vi "Check DAQmx Installed.vi"() -> (3 "DAQmx Installed?":bool)   [LabVIEW 2019]
doc: "Returns TRUE if DAQmx is installed in the system, FALSE otherwise."
uses:
  <vilib>/Utility/sysdir.llb/System Directory Type.ctl
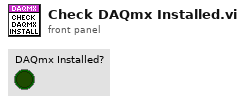
[diagram p1: front panel]
types:
  T1 = typedef "System Directory Type.ctl" = i32
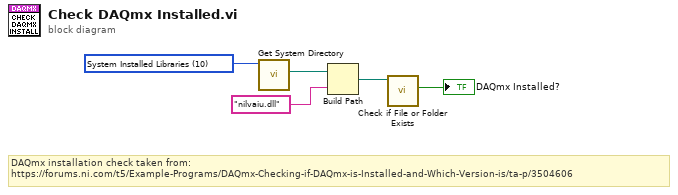
[diagram p0: block diagram]
diagram:
  w5 = T1 10 items=["User Home"=0, "User Desktop"=1, "User Documents"=2, "User Application Data"=3, "User Preferences"=4, "User Temporary"=5, "Public Documents"=6, "Public Application Data"=7, "Public Preferences"=8, "Public Cache"=13, "System Core Libraries"=9, "System Installed Libraries"=10, "Application Files"=11, "Boot Volume Root"=12] ("system directory type")
  # "DAQmx installation check taken from:\nhttps://forums.ni.com/t5/Example-Programs/DAQmx-Checking-if-DAQmx-is-Installed-and-Which-Version-is/ta-p/3504606"
  n1 = call <vilib>:"Get System Directory.vi"("system directory type"=w5) -> ("system directory"=w4:path)  [unwired: 10 in]
  n2 = Build Path(base path=w4, name or relative path="nilvaiu.dll") -> (appended path=w2:path)
  n3 = call <vilib>:"Check if File or Folder Exists.vi"("path"=w2) -> ("file or folder exists?"=→"DAQmx Installed?":bool)  [unwired: 8 in, 2 out]
